vi "Host_Report_Viewer.vi"(8 "error in (no error)":errorcluster={"status"=FALSE, "code"=0, "source"="\"\""}, 10 "report path/index":string, 11 "Run ID":string) -> (0 "error out":errorcluster={"status"=FALSE, "code"=0, "source"="\"\""}, 2 "status ok":bool, 3 "Rendered report summary":string)   [LabVIEW 2026]
doc: "INTENT: Browse completed report records. LOGIC: Filter run/step/cycle results and export copies; never modify source records."
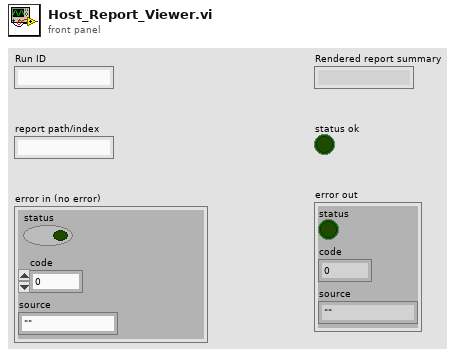
[diagram p1: front panel]
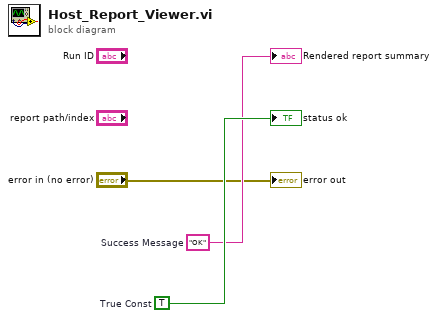
[diagram p0: block diagram]
diagram:
  w3 = TRUE  # True Const
  w2 = "OK"  # Success Message
  "Rendered report summary" <- w2
  "status ok" <- w3
  "error out" <- "error in (no error)"
